vi "VIH - VI Doc Editor #2 - Build Control Tree - Get GenObject Info.vi"(11 "Gen Refnum":refnum<vi>) -> (1 "Info":T1, 2 "Tree data":T2, 3 "dup Gen Refnum":refnum<vi>)   [LabVIEW 2014]
doc: "::: VI Helpeks :::\nCopyright (c) 2000-2026 Konstantin Shifershteyn. All rights reserved."
uses:
  VIH - VI Doc Editor #2 Typedef - Info Cluster.ctl
panel:
  # "VI Helpeks\nCopyright (c) 2012-2026 Konstantin Shifershteyn"
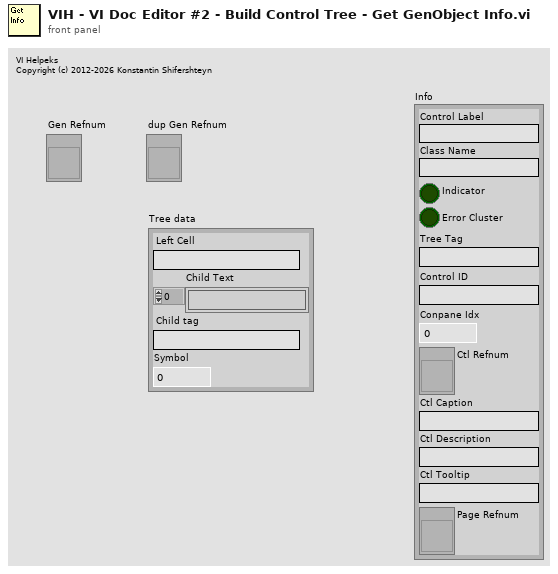
[diagram p1: front panel]
types:
  T1 = typedef "VIH - VI Doc Editor #2 Typedef - Info Cluster.ctl" = cluster{"Control Label":string, "Class Name":string, "Indicator":bool, "Error Cluster":bool, "Tree Tag":string, "Control ID":string, "Conpane Idx":i32, "Ctl Refnum":refnum<vi>, "Ctl Caption":string, "Ctl Description":string, "Ctl Tooltip":string, "Page Refnum":refnum<vi>}
  T2 = cluster{"Left Cell":string, "Child Text":string[], "Child tag":string, "Symbol":i32}
  T3 = enum16{"nop", "Init", "get index", "get symbols"}
  T4 = cluster{"Has Caption":bool, "Caption":string, "Description":string, "Tip Strip":string}
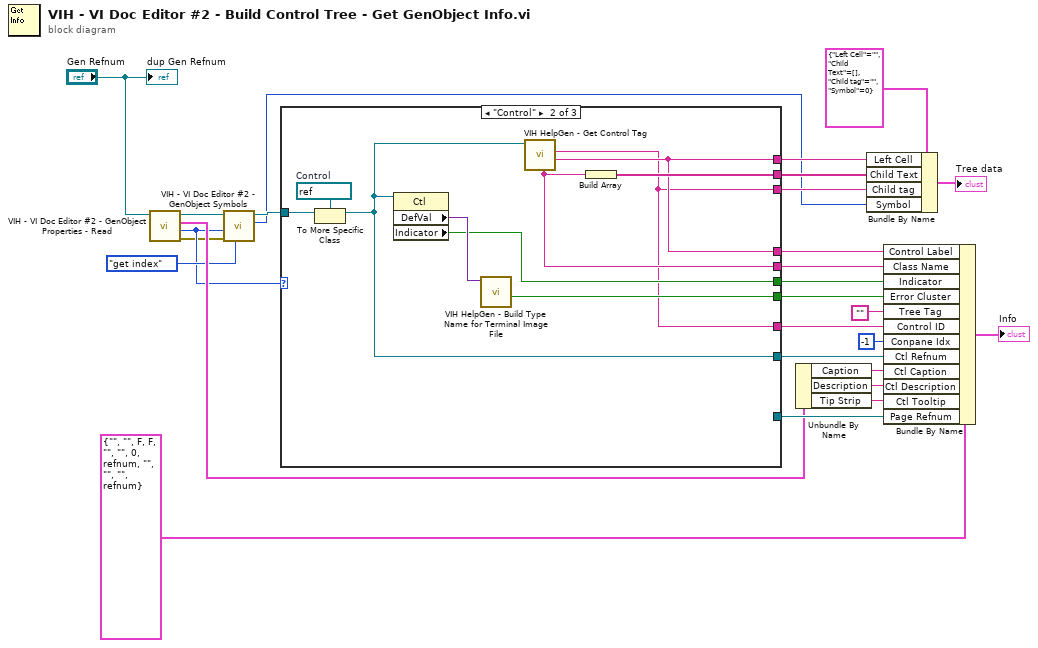
[diagram p0: block diagram]
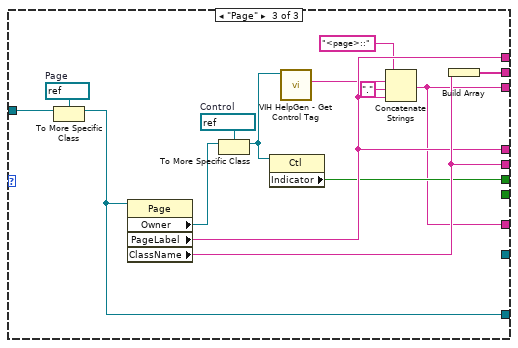
[diagram p3: hidden frame]
diagram:
  n1 = call "VIH - VI Doc Editor #2 - GenObject Properties - Read.vi"("Gen Refnum"="Gen Refnum") -> ("error out"=w2:errorcluster, "type"=w3:enum16{"<Invalid>", "Control", "Page"}, "Props"=w7:T4, "dup Gen Refnum"=w5:refnum<vi>)  [unwired: 7 in]
  n2 = call "VIH - VI Doc Editor #2 - GenObject Symbols.vi"("cmd (nop)"=T3."get index", "error in"=w2, "type"=w3, "Gen Refnum"=w5) -> ("Symbol Index"=w1:i32, "dup Gen Refnum"=w4:refnum<vi>)  [unwired: 4 in, 2 out]
  n3 = case shown="\"Control\"" w3 {
    tunnel: [_ w36 w47] -> w24
    tunnel: [_ w37 w46] -> w23
    tunnel: [_ w31 w44] -> w22
    tunnel: [_ w36 w47] -> w21
    tunnel: [_ w35 w48] -> w20
    tunnel: [_ w33 _] -> w19
    tunnel: [_ w32 w45] -> w18
    tunnel: [_ w31 w44] -> w16
    tunnel: [_ w28 _] -> w14
    tunnel: w4 -> [_ w29 w50]
    tunnel: [_ _ w49] -> w13
    frame "<Invalid>" {
    }
    frame "Control" {
      w30 = refnum<vi> refnum  # Control
      n4 = To More Specific Class(target class=w30, reference=w29) -> (specific class reference=w28:refnum<vi>)  [unwired: 1 in, 1 out]
      n5 = property class="Ctl"(reference=w28) -> ("DefVal"=w34:variant, "Indicator"=w32:bool)  [unwired: 1 in, 2 out]
      n6 = call "VIH HelpGen - Build Type Name for Terminal Image File.vi"("variant"=w34) -> ("Error Cluster"=w33:bool)  [unwired: 9 in, 1 out]
      n7 = call "VIH HelpGen - Get Control Tag.vi"("Ctl Refnum"=w28) -> ("Label"=w36:string, "Control Tag"=w31:string, "Class Name"=w35:string)  [unwired: 5 in, 3 out]
      n8 = Build Array(w35) -> (w37:string[])
    }
    frame "Page" {
      w42 = refnum<vi> refnum  # Control
      w51 = refnum<vi> refnum  # Page
      n9 = To More Specific Class(target class=w51, reference=w50) -> (specific class reference=w49:refnum<vi>)  [unwired: 1 in, 1 out]
      n10 = property class="Page"(reference=w49) -> ("Owner"=w43:refnum<vi>, "PageLabel"=w47:string, "ClassName"=w48:string)  [unwired: 1 in, 2 out]
      n11 = To More Specific Class(target class=w42, reference=w43) -> (specific class reference=w40:refnum<vi>)  [unwired: 1 in, 1 out]
      n12 = property class="Ctl"(reference=w40) -> ("Indicator"=w45:bool)  [unwired: 1 in, 2 out]
      n13 = call "VIH HelpGen - Get Control Tag.vi"("Ctl Refnum"=w40) -> ("Control Tag"=w39:string)  [unwired: 5 in, 5 out]
      n14 = Concatenate Strings("<page>::", w39, "." ("string"), w47) -> (w44:string)
      n15 = Build Array(w48) -> (w46:string[])
    }
  }
  n16 = Unbundle By Name(w7) -> ("Caption"=w10:string, "Description"=w9:string, "Tip Strip"=w8:string)
  n17 = Bundle By Name(cluster=T2 {"Left Cell"="", "Child Text"=[], "Child tag"="", "Symbol"=0} ("Tree data"), "Left Cell"=w24, "Child Text"=w23, "Child tag"=w22, "Symbol"=w1) -> (→"Tree data":T2)
  n18 = Bundle By Name(cluster=T1 {"Control Label"="", "Class Name"="", "Indicator"=FALSE, "Error Cluster"=FALSE, "Tree Tag"="", "Control ID"="", "Conpane Idx"=0, "Ctl Refnum"=refnum, "Ctl Caption"="", "Ctl Description"="", "Ctl Tooltip"="", "Page Refnum"=refnum} ("Info"), "Control Label"=w21, "Class Name"=w20, "Indicator"=w18, "Error Cluster"=w19, "Tree Tag"="", "Control ID"=w16, "Conpane Idx"=-1, "Ctl Refnum"=w14, "Ctl Caption"=w10, "Ctl Description"=w9, "Ctl Tooltip"=w8, "Page Refnum"=w13) -> (→"Info":T1)
  "dup Gen Refnum" <- "Gen Refnum"
